vi "Path Usage Values.vi"(0 "absolute default":path=path "C:/WireLint/default.txt", 5 "relative default":path=path "WireLint/default.txt", 11 "error in":errorcluster) -> (15 "error out":errorcluster)   [LabVIEW 2024]
doc: "Exposes path literals and defaults for static analysis without file operations."
panel:
  out "relative default text":string
  out "absolute default text":string
  out "fixed empty text":string
  out "relative text":string
  out "absolute text":string
  out "ordinary empty text":string
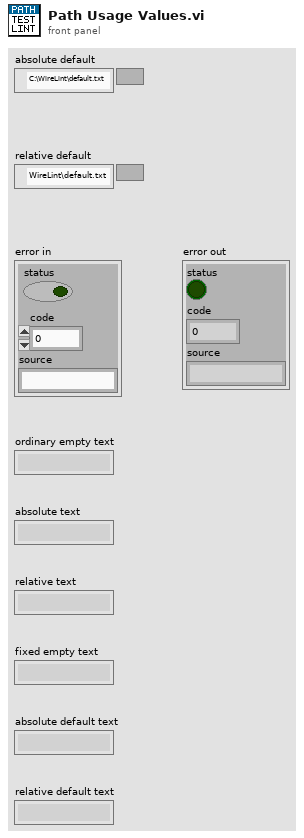
[diagram p1: front panel]
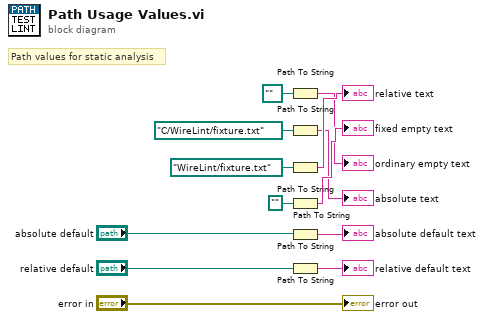
[diagram p0: block diagram]
diagram:
  # "Path values for static analysis"
  n1 = Path To String(path=path "" ("ordinary empty path")) -> (string=→"ordinary empty text":string)
  n2 = Path To String(path=path "C:/WireLint/fixture.txt" ("absolute path")) -> (string=→"absolute text":string)
  n3 = Path To String(path=path "WireLint/fixture.txt" ("relative path")) -> (string=→"relative text":string)
  n4 = Path To String(path=path "") -> (string=→"fixed empty text":string)
  n5 = Path To String(path="absolute default") -> (string=→"absolute default text":string)
  n6 = Path To String(path="relative default") -> (string=→"relative default text":string)
  "error out" <- "error in"
